vi "PostCall.vi"(8 "error in (no error)":errorcluster, 11 "LabVIEW Web Service Request":refnum<class "Web Request.lvclass"> caption="LabVIEW Web Service Request in") -> (0 "error out":errorcluster)   [LabVIEW 2017]
uses:
  <vilib>/wsapi/Web Request.lvclass
  ITool/ITool.lvclass
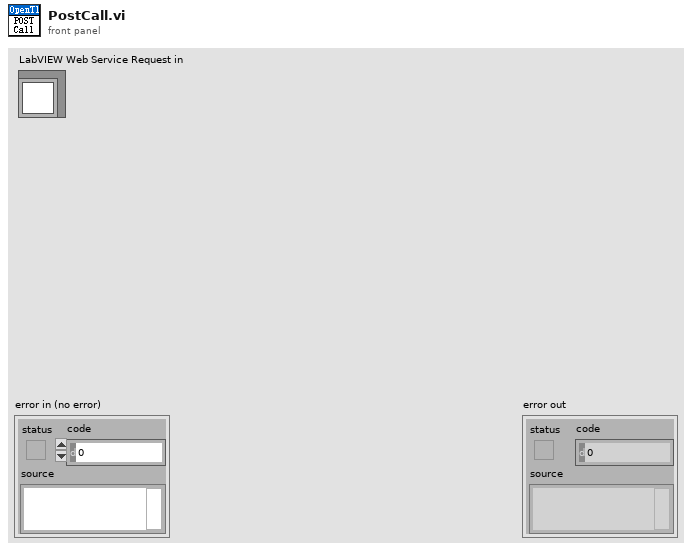
[diagram p1: front panel]
types:
  T1 = cluster{"jsonrpc":string, "id":string, "function":string, "arguments":variant}
  T2 = cluster{"jsonrpc":string, "result":variant, "id":string, "JsonRPCHttpResponseBodyError":cluster{"code":i32, "message":string}}
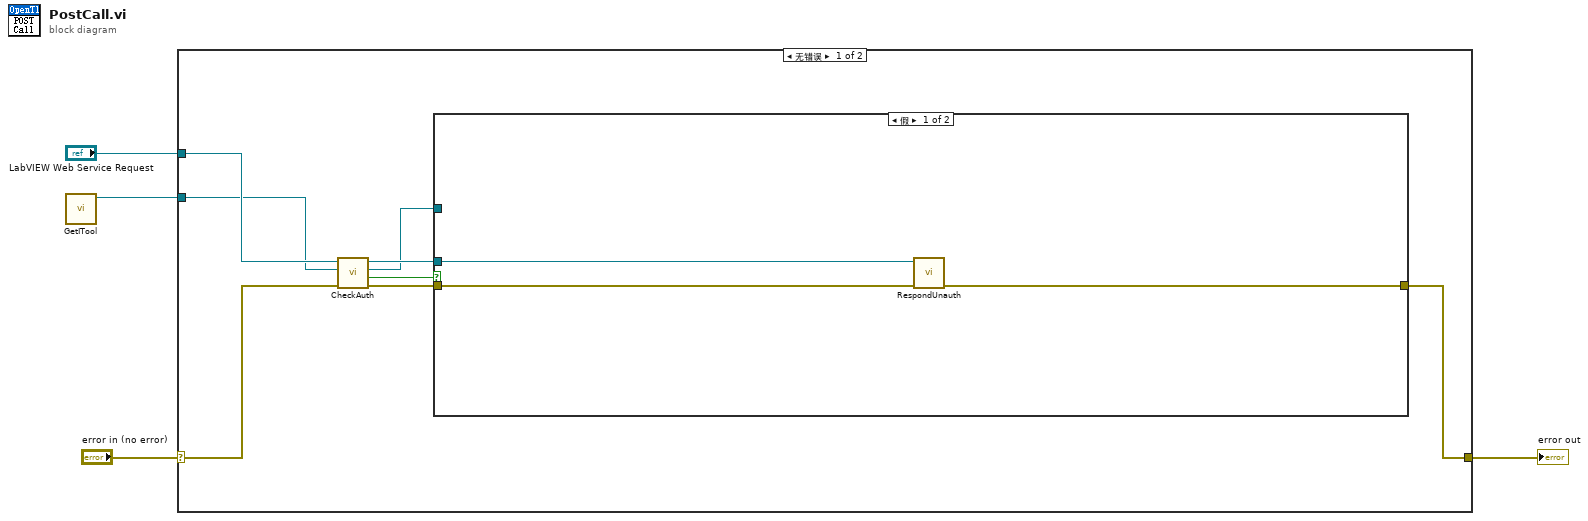
[diagram p0: block diagram]
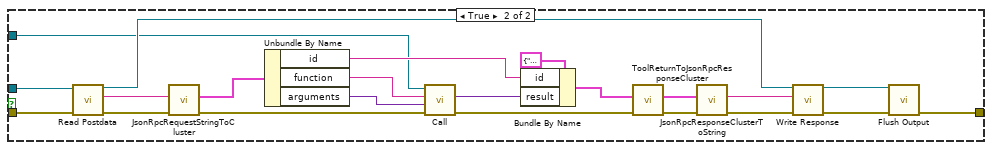
[diagram p2: hidden frame]
diagram:
  n1 = call "GetITool.vi"() -> ("ITool.lvclass out"=w1:refnum<class "ITool.lvclass">)  [unwired: 11 in]
  n2 = case shown="无错误" "error in (no error)" {
    selector: "error in (no error)" -> [w11 w38]
    tunnel: [w12 w38] -> w3
    tunnel: "LabVIEW Web Service Request" -> [w9 _]
    tunnel: w1 -> [w7 _]
    frame No Error {
      n3 = call "CheckAuth.vi"("error in (no error)"=w11, "ITool in"=w7, "LabVIEW Web Service Request"=w9) -> ("error out"=w10:errorcluster, "isAuthrized"=w6:bool, "ITool out"=w5:refnum<class "ITool.lvclass">, "LabVIEW Web Service Request out"=w8:refnum<class "Web Request.lvclass">)  [unwired: 5 in]
      n4 = case shown="假" w6 {
        tunnel: [w13 w19] -> w12
        tunnel: w10 -> [w15 w18]
        tunnel: w8 -> [w14 w17]
        tunnel: w5 -> [_ w16]
        frame False {
          n5 = call "RespondUnauth.vi"("error in (no error)"=w15, "LabVIEW Web Service Request"=w14) -> ("error out"=w13:errorcluster)  [unwired: 9 in]
        }
        frame True {
          n6 = call <vilib>:"Read Postdata.vi"("LabVIEW Web Service Request"=w17, "error in (no error)"=w18) -> ("LabVIEW Web Service Request out"=w26:refnum<class "Web Request.lvclass">, "postdata"=w37:string, "error out"=w36:errorcluster)  [unwired: 11 in]
          n7 = call "JsonRpcRequestStringToCluster.vi"("error in (no error)"=w36, "JsonRpcHttpRequestBodyString"=w37) -> ("error out"=w32:errorcluster, "JsonRPCHttpRequestBody"=w35:T1)  [unwired: 8 in]
          n8 = Unbundle By Name(w35) -> ("id"=w31:string, "function"=w34:string, "arguments"=w33:variant)
          n9 = call-dynamic "Call.vi"("error in (no error)"=w32, "Arguments"=w33, "Function"=w34, "Tool in"=w16) -> ("error out"=w28:errorcluster, "Result"=w29:variant)  [unwired: 5 in, 1 out]
          n10 = Bundle By Name(cluster=cluster{"id":string, "result":variant} {"id"="", "result"=variant} ("ToolReturn"), "id"=w31, "result"=w29) -> (w27:cluster{"id":string, "result":variant})
          n11 = call "ToolReturnToJsonRpcResponseCluster.vi"("error in (no error)"=w28, "ToolReturn"=w27) -> ("error out"=w24:errorcluster, "JsonRPCHttpResponseBody"=w25:T2)  [unwired: 8 in]
          n12 = call "JsonRpcResponseClusterToString.vi"("error in (no error)"=w24, "JsonRPCHttpResponseBody"=w25) -> ("error out"=w23:errorcluster, "JsonRPCHttpResonseBodyString"=w22:string)  [unwired: 8 in]
          n13 = call <vilib>:"Write Response.vi"("LabVIEW Web Service Request"=w26, "response string"=w22, "error in (no error)"=w23) -> ("LabVIEW Web Service Request out"=w20:refnum<class "Web Request.lvclass">, "error out"=w21:errorcluster)  [unwired: 11 in]
          n14 = call <vilib>:"Flush Output.vi"("LabVIEW Web Service Request"=w20, "error in (no error)"=w21) -> ("error out"=w19:errorcluster)  [unwired: 12 in, 1 out]
        }
      }
    }
    frame Error {
    }
  }
  "error out" <- w3
